vi "Append Price.vi"(10 "new price":dbl, 11 "prices":dbl[](array[numeric])) -> (3 "prices out":dbl[](array[numeric]))   [LabVIEW 2020, in "Full Featured MCP Server.lvlib"]
doc: "Appends a new price to the history of one stock and drops the oldest prices beyond two hours, so the history cannot grow without limit."
uses:
  Full Featured MCP Server.lvlib
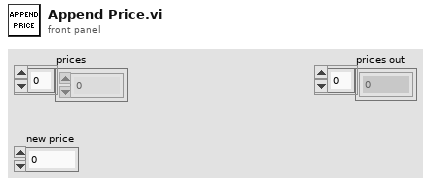
[diagram p1: front panel]
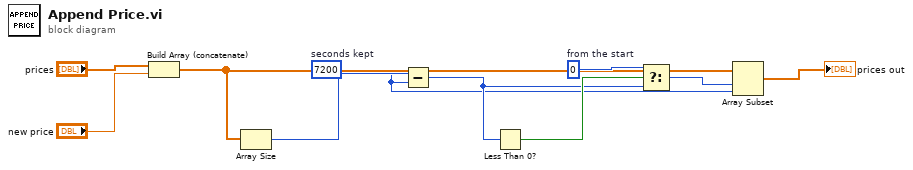
[diagram p0: block diagram]
diagram:
  w8 = 0  # from the start
  w3 = 7200  # seconds kept
  n1 = Build Array (concatenate)("prices", "new price") -> (w4:dbl[])
  n2 = Array Size(array=w4) -> (size(s)=w5:i32)
  n3 = Subtract(x=w5, y=w3) -> (x-y=w6:i32)
  n4 = Less Than 0?(x=w6) -> (x < 0?=w7:bool)
  n5 = Select(t=w8, s=w7, f=w6) -> (s? t:f=w9:i32)
  n6 = Array Subset(array=w4, index=w9, length=w3) -> (→"prices out":dbl[])
